vi "Initialise.vi"(6 "SubPanelReference":refnum<vi>, 7 "InitialRoute":string, 8 "error in (no error)":errorcluster, 11 "Routes":T1[](array[typedef])) -> (0 "error out":errorcluster, 3 "Navigator out":refnum<class "Navigator.lvclass">)   [LabVIEW 2024, in "Navigator.lvclass"]
doc: "Initialise Navigator class."
uses:
  Navigator.lvclass
  Route.ctl
  NavigatableView/NavigatableView.lvclass
  NavigatorEvents.ctl
  Navigator.lvclass/Navigator.ctl
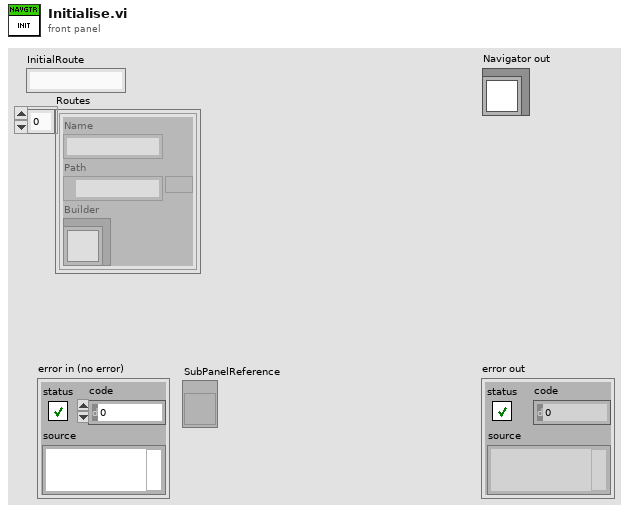
[diagram p1: front panel]
types:
  T1 = typedef "Navigator.lvclass/Route.ctl" = cluster{"Name":string, "Path":path, "Builder":refnum<class "NavigatableView.lvclass">}
  T2 = typedef "Navigator.lvclass/NavigatorEvents.ctl" = cluster{"go":refnum<user-event>, "push":refnum<user-event>, "pop":refnum<user-event>}
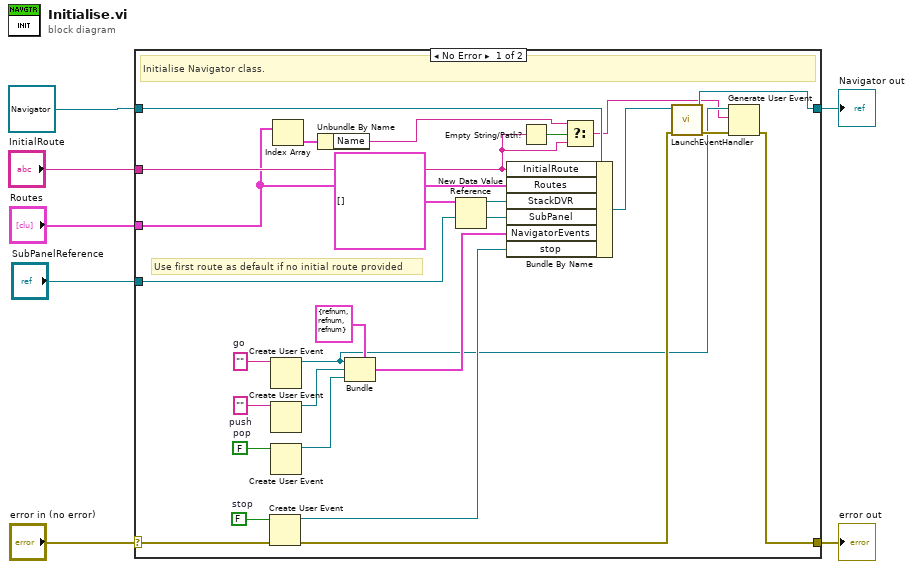
[diagram p0: block diagram]
diagram:
  n1 = case shown="No Error" "error in (no error)" {
    selector: "error in (no error)" -> [w23 w35]
    tunnel: [w18 w35] -> w6
    tunnel: [w16 w34] -> w4
    tunnel: refnum<class "Navigator.lvclass"> refnum ("Navigator in") -> [w26 w34]
    tunnel: "InitialRoute" -> [w12 _]
    tunnel: "SubPanelReference" -> [w22 _]
    tunnel: "Routes" -> [w10 _]
    frame No Error {
      w27 = FALSE  # stop
      w32 = ""  # push
      w33 = ""  # go
      w31 = FALSE  # pop
      # "Use first route as default if no initial route provided"
      # "Initialise Navigator class."
      n2 = Create User Event(user event datatype=w27, error in=w23) -> (user event=w24:refnum<user-event>, error out=w20:errorcluster)
      n3 = Create User Event(user event datatype=w33) -> (user event=w17:refnum<user-event>)  [unwired: 1 in, 1 out]
      n4 = Create User Event(user event datatype=w32) -> (user event=w30:refnum<user-event>)  [unwired: 1 in, 1 out]
      n5 = Create User Event(user event datatype=w31) -> (user event=w29:refnum<user-event>)  [unwired: 1 in, 1 out]
      n6 = Index Array(array=w10) -> (element=w9:T1)  [unwired: 1 in]
      n7 = Unbundle By Name(w9) -> ("Name"=w8:string)
      n8 = Bundle(cluster=T2 {"go"=refnum, "push"=refnum, "pop"=refnum} ("output cluster"), "go"=w17, "push"=w30, "pop"=w29) -> (w25:T2)
      n9 = New Data Value Reference(data value=T1[] [] ("Stack")) -> (data value reference=w14:refnum<data-value>)  [unwired: 1 in, 1 out]
      n10 = Bundle By Name(cluster=w26, "InitialRoute"=w12, "Routes"=w10, "StackDVR"=w14, "SubPanel"=w22, "NavigatorEvents"=w25, "stop"=w24) -> (w21:refnum<class "Navigator.lvclass">)
      n11 = Empty String/Path?(string/path=w12) -> (empty?=w13:bool)
      n12 = Select(t=w8, s=w13, f=w12) -> (s? t:f=w11:string)
      n13 = call "LaunchEventHandler.vi"("error in (no error)"=w20, "Navigator in"=w21) -> ("error out"=w19:errorcluster, "Navigator out"=w16:refnum<class "Navigator.lvclass">)  [unwired: 8 in]
      n14 = Generate User Event(user event=w17, event data cluster=w11, error in=w19) -> (error out=w18:errorcluster)  [unwired: 1 in, 1 out]
    }
    frame Error {
    }
  }
  "error out" <- w6
  "Navigator out" <- w4
